vi "Initialize NodeBrowserWF.vi"(7 "Generate?":bool, 8 "error in (no error)":errorcluster, 9 "Output Channels":T2[](array[typedef]) {"Data Type" items=["Signed", "Unsigned", "IEEE Float"]}, 10 "Node Pointer":T1, 11 "NodeBrowserRefs":refnum<k24>[](array[refnum])) -> (0 "error out":errorcluster, 2 "Node Pointer":T1, 3 "NodeBrowserRefs":refnum<k24>[](array[refnum]))   [LabVIEW 2015, in "Protection and Rolling Counter Addon System Explorer.lvlib"]
uses:
  Protection and Rolling Counter Addon System Explorer.lvlib
  Shared/Types/InputChannelConfiguration.ctl
  <vilib>/NI Veristand/Custom Device API/Custom Device Pointer.ctl
  NationalInstruments.VeriStand.SystemStorage
  NationalInstruments.VeriStand.SystemStorageUI
  NationalInstruments.VeriStand
  Shared/Protection and Rolling Counter Addon Shared.lvlib
  <vilib>/NI Veristand/Custom Device API/Custom Device API.lvlib
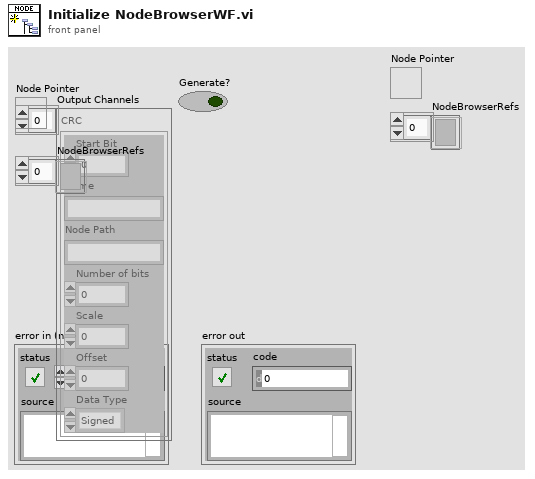
[diagram p1: front panel]
types:
  T1 = typedef "Custom Device API.lvlib/Custom Device Pointer.ctl" = refnum<k24>
  T2 = typedef "Protection and Rolling Counter Addon Shared.lvlib/InputChannelConfiguration.ctl" = cluster{"Start Bit":i32, "Name":string, "Node Path":string, "Number of bits":i32, "Scale":dbl, "Offset":dbl, "Data Type":u32}
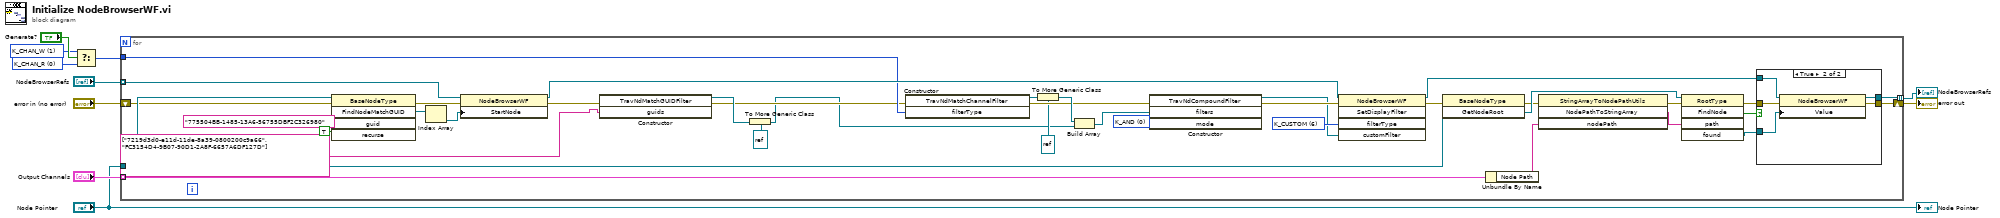
[diagram p0: block diagram]
diagram:
  w2 = u8 0 items=["K_CHAN_R", "K_CHAN_W", "K_CHAN_VOLT", "K_CHAN_FAULT"] ("filterType")
  w3 = u8 1 items=["K_CHAN_R", "K_CHAN_W", "K_CHAN_VOLT", "K_CHAN_FAULT"] ("filterType")
  n1 = Select(t=w3, s="Generate?", f=w2) -> (s? t:f=w4:u8)
  n2 = for {
    tunnel: "NodeBrowserRefs" -> [w48] mode=indexing
    tunnel: [w39] -> w6 mode=indexing
    tunnel: "Node Pointer" -> [w32]
    shift-right: [w38] -> w10
    shift-left: "error in (no error)" -> [w29]
    tunnel: "Output Channels" -> [w37] mode=indexing
    tunnel: w4 -> [w16]
    w25 = 0 items=["K_AND", "K_OR"] ("mode")
    w35 = u8 6 items=["K_CHAN_R", "K_CHAN_W", "K_CHAN_RW", "K_CHAN_VOLT", "K_CHAN_FAULT", "K_ALL", "K_CUSTOM", "K_CHAN_R_VIS", "K_CHAN_W_VIS", "K_CHAN_RW_VIS", "K_CHAN_VOLT_VIS", "K_CHAN_FAULT_VIS", "K_WAVE", "K_WAVE_VIS", "K_WAVE_DBL", "K_WAVE_CDB", "K_WAVE_DBL_VIS", "K_WAVE_CDB_VIS"] ("filterType")
    n3 = invoke class="BaseNodeType" method="FindNodeMatchGUID"(reference=w32, error in=w29, "guid"="775504BB-1485-13A6-56755DBF2C326980", "recurse"=TRUE) -> (error out=w28:errorcluster, "FindNodeMatchGUID"=w31:refnum<k24>[])  [unwired: 1 in, 3 out]
    n4 = Index Array(array=w31) -> (element=w30:refnum<k24>)  [unwired: 1 in]
    n5 = property class="NodeBrowserWF"(reference=w48, error in=w28, "StartNode"=w30) -> (reference out=w17:refnum<k24>, error out=w33:errorcluster)
    n6 = constructor class="TravNdMatchGUIDFilter"(error in=w33, "guids"=string[] ["7219d3d0-e11d-11de-8a39-0800200c9a66", "FC3154D4-9B07-90D1-2A8F-6657A6DF127D"]) -> (reference out=w14:refnum<k24>, error out=w12:errorcluster)  [unwired: 2 in, 2 out]
    n7 = To More Generic Class(target class=refnum<k24> refnum, reference=w14) -> (generic class reference=w11:refnum<k24>)
    n8 = constructor class="TravNdMatchChannelFilter"(error in=w12, "filterType"=w16) -> (reference out=w19:refnum<k24>, error out=w21:errorcluster)  [unwired: 2 in, 2 out]
    n9 = To More Generic Class(target class=refnum<k24> refnum, reference=w19) -> (generic class reference=w24:refnum<k24>)
    n10 = Build Array(w24, w11) -> (w23:refnum<k24>[])
    n11 = constructor class="TravNdCompoundFilter"(error in=w21, "filters"=w23, "mode"=w25) -> (reference out=w18:refnum<k24>, error out=w22:errorcluster)  [unwired: 2 in, 3 out]
    n12 = invoke class="NodeBrowserWF" method="SetDisplayFilter"(reference=w17, error in=w22, "filterType"=w35, "customFilter"=w18) -> (reference out=w47:refnum<k24>, error out=w41:errorcluster)  [unwired: 1 in, 3 out]
    n13 = invoke class="BaseNodeType" method="GetNodeRoot"(reference=w32, error in=w41) -> (error out=w45:errorcluster, "GetNodeRoot"=w46:refnum<k24>)  [unwired: 1 in, 1 out]
    n14 = Unbundle By Name(w37) -> ("Node Path"=w36:string)
    n15 = invoke class="StringArrayToNodePathUtils" method="NodePathToStringArray"(error in=w45, "nodePath"=w36) -> (error out=w43:errorcluster, "NodePathToStringArray"=w44:string[])  [unwired: 2 in, 2 out]
    n16 = invoke class="RootType" method="FindNode"(reference=w46, error in=w43, "path"=w44) -> (error out=w40:errorcluster, "FindNode"=w34:bool, "found"=w42:refnum<k24>)  [unwired: 2 in, 2 out]
    n17 = case shown="True" w34 {
      tunnel: w47 -> [w49 w55]
      tunnel: w42 -> [_ w54]
      tunnel: w40 -> [w50 w53]
      tunnel: [w49 w52] -> w39
      tunnel: [w50 w51] -> w38
      frame False {
      }
      frame True {
        n18 = property class="NodeBrowserWF"(reference=w55, error in=w53, "Value"=w54) -> (reference out=w52:refnum<k24>, error out=w51:errorcluster)
      }
    }
  }
  "error out" <- w10
  "NodeBrowserRefs" <- w6
  "Node Pointer" <- "Node Pointer"
